vi "Reserve SCOPE Session.vi"(7 "Simulate":bool, 8 "error in (no error)":errorcluster, 9 "Measurement Configuration In":T1={"Start Frequency"=100.0, "Frequency Steps"=10.0, "Stop Frequency"=1000000.0, "Amplitude"=1.0, "Timing (ms)"=0, "Vin_signal"="Vin_signal", "filter_pins"="Vin_measure"} {"Stop Frequency" format="%#_6p"; "Frequency Steps" format="%#_6p"; "Start Frequency" format="%#_6p"}, 11 "Measurement Context":refnum<class "MeasurementContext.lvclass">) -> (0 "error out":errorcluster, 1 "Measurement Configuration Out":T1={"Start Frequency"=100.0, "Frequency Steps"=10.0, "Stop Frequency"=1000000.0, "Amplitude"=1.0, "Timing (ms)"=0, "Vin_signal"="Vin_signal", "filter_pins"="Vin_measure"} {"Stop Frequency" format="%#_6p"; "Frequency Steps" format="%#_6p"; "Start Frequency" format="%#_6p"}, 2 "Session":T2, 3 "Measurement Context out":refnum<class "MeasurementContext.lvclass">, 5 "scope_out":refnum<k15>)   [LabVIEW 2023, in "LabVIEW Bodeplot Summit.lvlib"]
doc: "Reserve Runtime Session for Scope Channels"
uses:
  LabVIEW Bodeplot Summit.lvlib
  <vilib>/MeasurementLink/MeasurementLink Measurement Server/Classes/MeasurementContext/MeasurementContext.lvclass
  Measurement Configuration.ctl
  Session Info.ctl
  <vilib>/gRPC/LabVIEW gRPC Library/Shared/grpcId.ctl
  <vilib>/MeasurementLink/MeasurementLink Session Management Client/RPC Messages/ni_measurementlink_sessionmanagement_v1_ReserveSessionsResponse.ctl
  <vilib>/MeasurementLink/MeasurementLink Session Management Client/RPC Messages/ni_measurementlink_sessionmanagement_v1_SessionInformation.ctl
  <vilib>/MeasurementLink/MeasurementLink Session Management Client/RPC Messages/nidevice_grpc_Session.ctl
  <vilib>/MeasurementLink/MeasurementLink Session Management Client/RPC Messages/ni_measurementlink_sessionmanagement_v1_ChannelMapping.ctl
  <vilib>/MeasurementLink/MeasurementLink Session Management Client/RPC Messages/ni_measurementlink_sessionmanagement_v1_ReserveSessionsRequest.ctl
  <vilib>/MeasurementLink/MeasurementLink Session Management Client/RPC Messages/ni_measurementlink_PinMapContext.ctl
  <vilib>/MeasurementLink/MeasurementLink Discovery Client/RPC Messages/ni_measurementlink_discovery_v1_ServiceLocation.ctl
  <vilib>/MeasurementLink/MeasurementLink Discovery Client/RPC Messages/ni_measurementlink_discovery_v1_ResolveServiceRequest.ctl
  <instrlib>/niScope/niScope gRPC Device Server.ctl
  <vilib>/MeasurementLink/MeasurementLink Measurement Server/MeasurementLink Measurement Server.lvlib
  <vilib>/MeasurementLink/MeasurementLink Session Management Client/MeasurementLink Session Management Client.lvlib
  <vilib>/MeasurementLink/MeasurementLink Discovery Client/MeasurementLink Discovery Client.lvlib
  <vilib>/gRPC/LabVIEW gRPC Library/grpc-lvsupport-release.lvlib
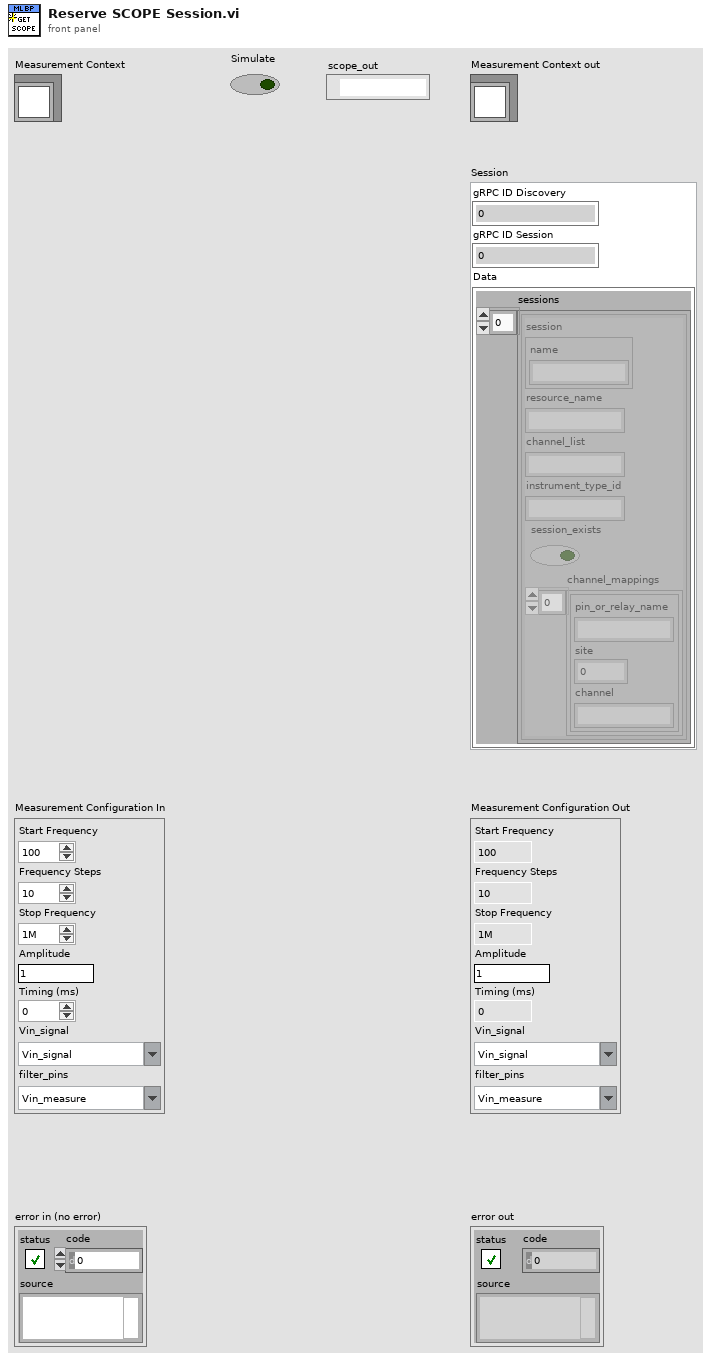
[diagram p1: front panel]
types:
  T1 = typedef "LabVIEW Bodeplot Summit.lvlib/Measurement Configuration.ctl" = cluster{"Start Frequency":dbl, "Frequency Steps":dbl, "Stop Frequency":dbl, "Amplitude":dbl, "Timing (ms)":u32, "Vin_signal":string, "filter_pins":string}
  T2 = typedef "LabVIEW Bodeplot Summit.lvlib/Session Info.ctl" = cluster{"gRPC ID Discovery":T3, "gRPC ID Session":T3, "Data":T4}
  T3 = typedef "grpc-lvsupport-release.lvlib/grpcId.ctl" = u64
  T4 = typedef "MeasurementLink Session Management Client.lvlib/ni_measurementlink_sessionmanagement_v1_ReserveSessionsResponse.ctl" = cluster{"sessions":T5[]}
  T5 = typedef "MeasurementLink Session Management Client.lvlib/ni_measurementlink_sessionmanagement_v1_SessionInformation.ctl" = cluster{"session":T6, "resource_name":string, "channel_list":string, "instrument_type_id":string, "session_exists":bool, "channel_mappings":T7[]}
  T6 = typedef "MeasurementLink Session Management Client.lvlib/nidevice_grpc_Session.ctl" = cluster{"name":string}
  T7 = typedef "MeasurementLink Session Management Client.lvlib/ni_measurementlink_sessionmanagement_v1_ChannelMapping.ctl" = cluster{"pin_or_relay_name":string, "site":i32, "channel":string}
  T8 = typedef "MeasurementLink Discovery Client.lvlib/ni_measurementlink_discovery_v1_ServiceLocation.ctl" = cluster{"location":string, "insecure_port":string, "ssl_authenticated_port":string}
  T9 = typedef "MeasurementLink Session Management Client.lvlib/ni_measurementlink_sessionmanagement_v1_ReserveSessionsRequest.ctl" = cluster{"pin_map_context":T10, "pin_or_relay_names":string[], "instrument_type_id":string, "timeout_in_milliseconds":i32}
  T10 = typedef "MeasurementLink Session Management Client.lvlib/ni_measurementlink_PinMapContext.ctl" = cluster{"pin_map_id":string, "sites":i32[]}
  T11 = typedef "MeasurementLink Measurement Server.lvlib/PinMapContext.ctl" = cluster{"pin_map_id":string, "sites":i32[]}
  T12 = typedef "MeasurementLink Discovery Client.lvlib/ni_measurementlink_discovery_v1_ResolveServiceRequest.ctl" = cluster{"provided_interface":string, "service_class":string}
  T13 = typedef "niScope gRPC Device Server.ctl" = cluster{"session name":string, "address (localhost)":string, "port (31763)":u32}
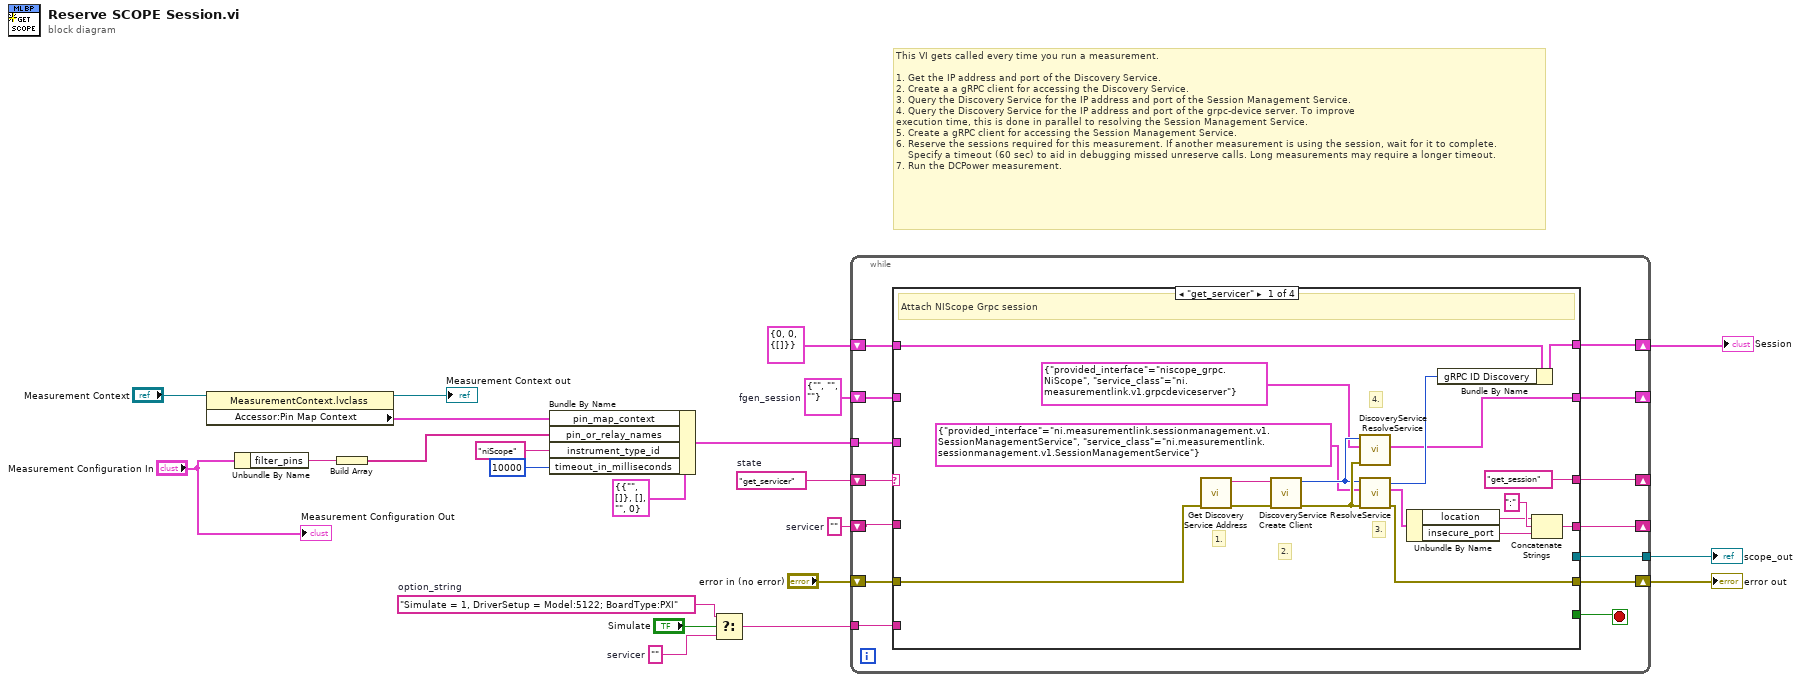
[diagram p0: block diagram]
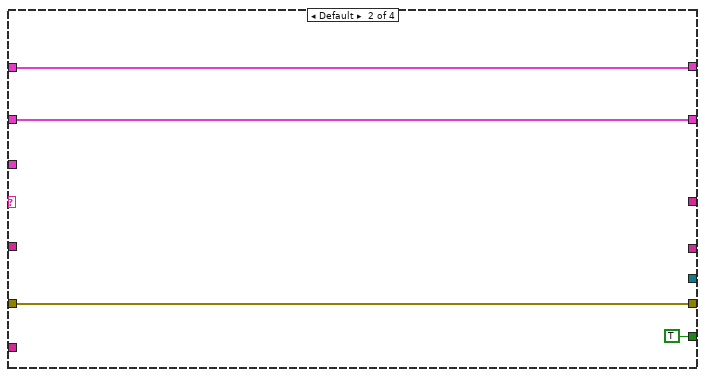
[diagram p2: hidden frame]
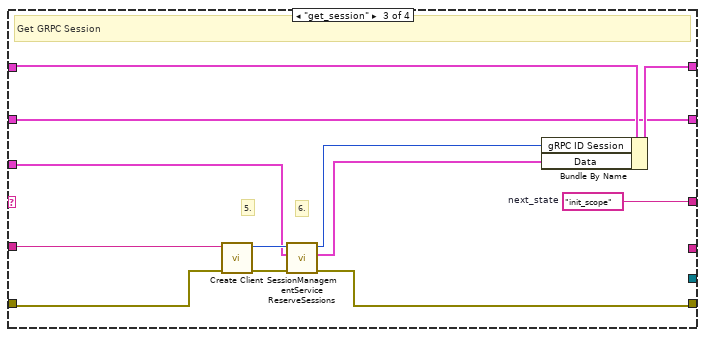
[diagram p3: hidden frame]
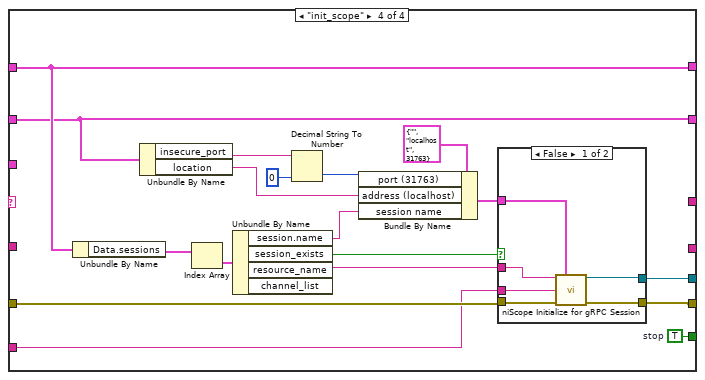
[diagram p4: hidden frame]
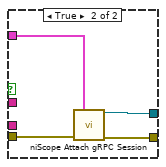
[diagram p5: hidden frame]
diagram:
  w5 = "Simulate = 1, DriverSetup = Model:5122; BoardType:PXI"  # option_string
  w4 = ""  # servicer
  w10 = T8 {"location"="", "insecure_port"="", "ssl_authenticated_port"=""}  # fgen_session
  w13 = ""  # servicer
  w16 = "get_servicer"  # state
  # "This VI gets called every time you run a measurement.\n\n1. Get the IP address and port of the Discovery Service.\n2. Create a a gRPC client for accessing the Discovery Service.\n3. Query the Discovery Service for the IP address and port of the Session Management Service.\n4. Query the Discovery Service for the IP address and port of the grpc-device server. To improve \nexecution time, this is done in parallel to resolving the Session Management Service.\n5. Create a gRPC client for accessing the Session Management Service.\n6. Reserve the sessions required for this measurement. If another measurement is using the session, wait for it to complete. \n    Specify a timeout (60 sec) to aid in debugging missed unreserve calls. Long measurements may require a longer timeout.\n7. Run the DCPower measurement."
  n1 = property class="MeasurementContext.lvclass"(reference="Measurement Context") -> (reference out=→"Measurement Context out":refnum<class "MeasurementContext.lvclass">, "Accessor:Pin Map Context"=w20:T11)  [unwired: 1 in, 1 out]
  n2 = Unbundle By Name("Measurement Configuration In") -> ("filter_pins"=w2:string)
  n3 = Build Array(w2) -> (w1:string[])
  n4 = Bundle By Name(cluster=T9 {"pin_map_context"={"pin_map_id"="", "sites"=[]}, "pin_or_relay_names"=[], "instrument_type_id"="", "timeout_in_milliseconds"=0} ("Request Data"), "pin_map_context"=w20, "pin_or_relay_names"=w1, "instrument_type_id"="niScope" ("Instrument Type Id"), "timeout_in_milliseconds"=10000) -> (w12:T9)
  n5 = Select(t=w5, s="Simulate", f=w4) -> (s? t:f=w3:string)
  n6 = while {
    shift-right: [w30] -> _
    shift-left: w16 -> [w36]
    shift-right: [w32] -> w11
    shift-left: T2 {"gRPC ID Discovery"=0, "gRPC ID Session"=0, "Data"={"sessions"=[]}} ("Session") -> [w33]
    shift-right: [w31] -> _
    shift-left: w13 -> [w29]
    shift-right: [w34] -> w8
    shift-left: "error in (no error)" -> [w35]
    tunnel: w12 -> [w28]
    shift-right: [w27] -> _
    shift-left: w10 -> [w26]
    tunnel: w3 -> [w25]
    tunnel: [w24] -> w9
    stop <- w23 stop-if-true
    n7 = case shown="\"get_servicer\"" w36 {
      tunnel: w35 -> [w48 w56 w67 w76]
      tunnel: [w47 w56 w62 w75] -> w34
      tunnel: w33 -> [w46 w58 w65 w87]
      tunnel: [w45 w58 w63 w87] -> w32
      tunnel: [w39 _ _ _] -> w31
      tunnel: ["get_session" _ w60 _] -> w30
      tunnel: w29 -> [_ _ w68 _]
      tunnel: w28 -> [_ _ w66 _]
      tunnel: [w37 w57 w59 w77] -> w27
      tunnel: w26 -> [_ w57 w59 w77]
      tunnel: w25 -> [_ _ _ w74]
      tunnel: [_ _ _ w73] -> w24
      tunnel: [_ TRUE _ w72] -> w23
      frame "get_servicer" {
        # "4."
        # "3."
        # "2."
        # "1."
        # "Attach NIScope Grpc session"
        n8 = call <vilib>:"Get Discovery Service Address.vi"("error in"=w48) -> ("error out"=w51:errorcluster, "address"=w52:string)  [unwired: 9 in]
        n9 = call <vilib>:"Create Client.vi"("error in"=w51, "address"=w52) -> ("error out"=w54:errorcluster, "gRPC ID Out"=w53:T3)  [unwired: 8 in]
        n10 = call <vilib>:"DiscoveryService ResolveService.vi"("error in"=w54, "Request Data"=T12 {"provided_interface"="niscope_grpc.NiScope", "service_class"="ni.measurementlink.v1.grpcdeviceserver"}, "gRPC ID"=w53) -> ("Response Data"=w37:T8)  [unwired: 6 in, 2 out]
        n11 = call <vilib>:"DiscoveryService ResolveService.vi"("error in"=w54, "Request Data"=T12 {"provided_interface"="ni.measurementlink.sessionmanagement.v1.SessionManagementService", "service_class"="ni.measurementlink.sessionmanagement.v1.SessionManagementService"}, "gRPC ID"=w53) -> ("error out"=w47:errorcluster, "Response Data"=w42:T8, "gRPC ID out"=w44:T3)  [unwired: 6 in]
        n12 = Unbundle By Name(w42) -> ("location"=w41:string, "insecure_port"=w40:string)
        n13 = Bundle By Name(cluster=w46, "gRPC ID Discovery"=w44) -> (w45:T2)
        n14 = Concatenate Strings(w41, ":" ("string"), w40) -> (w39:string)
      }
      frame Default {
      }
      frame "get_session" {
        w60 = "init_scope"  # next_state
        # "6."
        # "5."
        # "Get GRPC Session"
        n15 = call <vilib>:"Create Client.vi"("error in"=w67, "address"=w68) -> ("error out"=w70:errorcluster, "gRPC ID Out"=w69:T3)  [unwired: 8 in]
        n16 = call <vilib>:"SessionManagementService ReserveSessions.vi"("error in"=w70, "Request Data"=w66, "gRPC ID"=w69) -> ("error out"=w62:errorcluster, "Response Data"=w64:T4, "gRPC ID out"=w61:T3)  [unwired: 6 in]
        n17 = Bundle By Name(cluster=w65, "gRPC ID Session"=w61, "Data"=w64) -> (w63:T2)
      }
      frame "init_scope" {
        w72 = TRUE  # stop
        n18 = Unbundle By Name(w87) -> ("Data.sessions"=w88:T5[])
        n19 = Unbundle By Name(w77) -> ("insecure_port"=w84:string, "location"=w83:string)
        n20 = Index Array(array=w88) -> (element=w78:T5)  [unwired: 1 in]
        n21 = Unbundle By Name(w78) -> ("session.name"=w82:string, "session_exists"=w80:bool, "resource_name"=w86:string)  [unwired: 1 out]
        n22 = Decimal String To Number(string=w84, default (0L)=u32 0 ("Port (31763)")) -> (number=w85:u32)  [unwired: 1 in, 1 out]
        n23 = Bundle By Name(cluster=T13 {"session name"="", "address (localhost)"="localhost", "port (31763)"=31763} ("gRPC options"), "port (31763)"=w85, "address (localhost)"=w83, "session name"=w82) -> (w81:T13)
        n24 = case shown="False" w80 {
          tunnel: w76 -> [w90 w98]
          tunnel: w81 -> [w93 w97]
          tunnel: [w92 w96] -> w75
          tunnel: [w94 w95] -> w73
          tunnel: w86 -> [w91 _]
          tunnel: w74 -> [w89 _]
          frame False {
            n25 = call <instrlib>:"niScope Initialize for gRPC Session.vi"("resource name"=w91, "gRPC options"=w93, "option string"=w89, "error in"=w90) -> ("instrument handle"=w94:refnum<k15>, "error out"=w92:errorcluster)  [unwired: 10 in]
          }
          frame True {
            n26 = call <instrlib>:"niScope Attach gRPC Session.vi"("gRPC options"=w97, "error in"=w98) -> ("instrument handle"=w95:refnum<k15>, "error out"=w96:errorcluster)  [unwired: 12 in]
          }
        }
      }
    }
  }
  "error out" <- w8
  "scope_out" <- w9
  "Session" <- w11
  "Measurement Configuration Out" <- "Measurement Configuration In"
